vi "Toast With Multiple Actions.vi"(8 "error in":errorcluster) -> (0 "error out":errorcluster, 3 "Toast XML":string)   [LabVIEW 2026]
doc: "Distinguish clicks on the Accept button, Reject button and toast body. Inspect Activation.Arguments after each action. User Inputs is empty because the toast has no input field. Press Stop to close the example."
uses:
  ToastNotification/Activation.ctl
  ToastNotification/Argument.ctl
  PlugIns/UserEventActivationHandler/UserEventActivationHandler.lvclass
  PlugIns/UserEventActivationHandler/UserEventActivationHandler.lvclass/UserEventActivationHandler.ctl
  PlugIns/UserEventActivationHandler/Read Event Ref.vi
  ToastBuilder/ToastBuilder.lvclass
  ToastBuilder/Create ToastBuilder.vi
  ToastService/ToastService.lvclass
  ToastNotification/ToastNotification.lvlib
panel:
  out "error":errorcluster
  out "Activation":T1
  in  "stop":bool
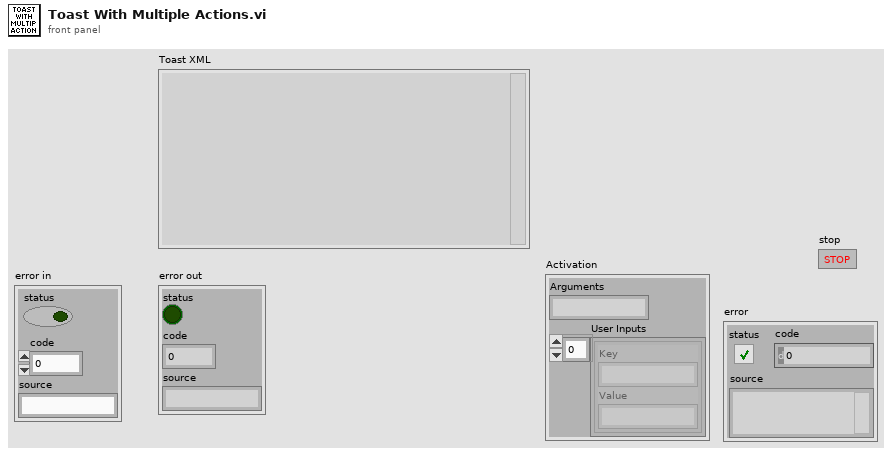
[diagram p1: front panel]
types:
  T1 = typedef "ToastNotification.lvlib/Activation.ctl" = cluster{"Arguments":string, "User Inputs":T2[]}
  T2 = typedef "ToastNotification.lvlib/Argument.ctl" = cluster{"Key":string, "Value":string}
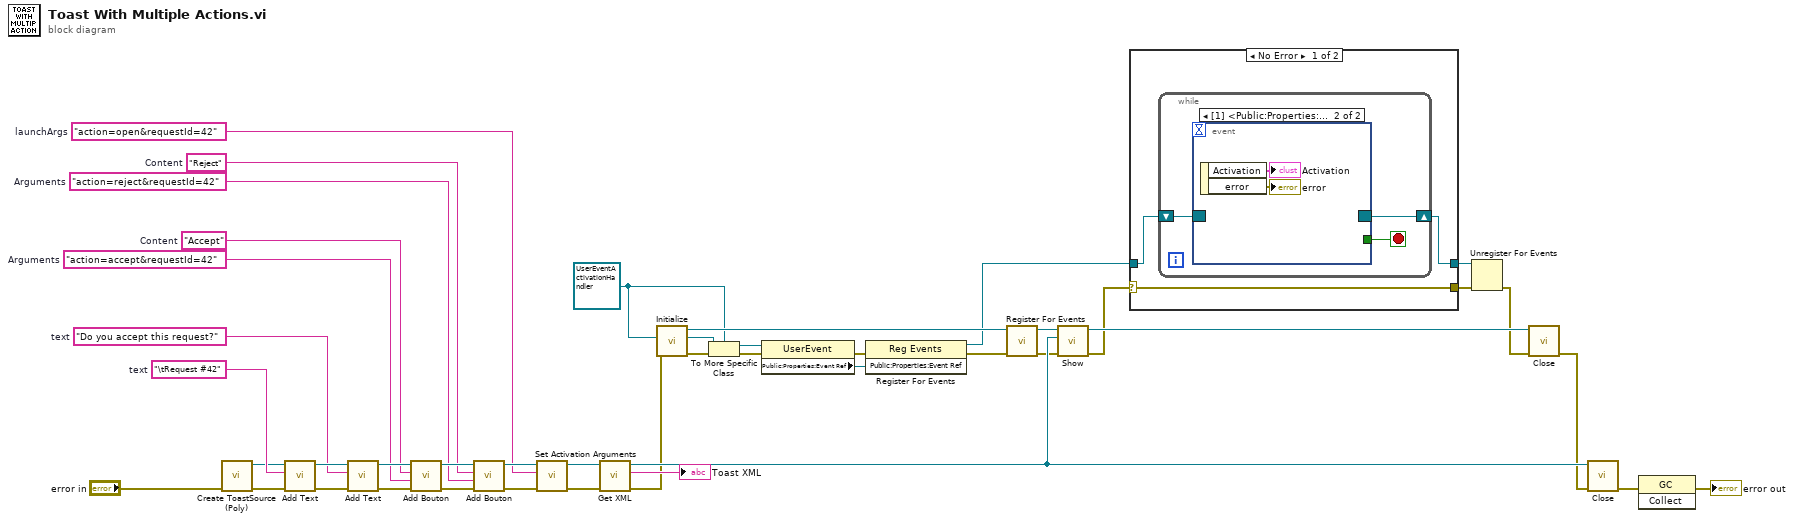
[diagram p0: block diagram]
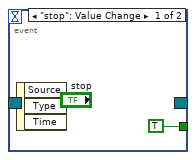
[diagram p2: hidden frame]
diagram:
  w1 = "action=open&requestId=42"  # launchArgs
  w10 = "action=reject&requestId=42"  # Arguments
  w9 = "Reject"  # Content
  w11 = "action=accept&requestId=42"  # Arguments
  w12 = "Accept"  # Content
  w13 = "Do you accept this request?"  # text
  w14 = "\tRequest #42"  # text
  w31 = refnum<class "UserEventActivationHandler.lvclass"> refnum
  n1 = call-poly "Create ToastSource (Poly).vi"("error in"="error in") -> ("error out"=w7:errorcluster, "ToastBuilder out"=w8:refnum<class "ToastBuilder.lvclass">)  [unwired: 9 in]
  n2 = call "Add Text.vi"("error in"=w7, "text"=w14, "ToastBuilder in"=w8) -> ("error out"=w19:errorcluster, "ToastBuilder out"=w20:refnum<class "ToastBuilder.lvclass">)  [unwired: 7 in]
  n3 = call "Add Text.vi"("error in"=w19, "text"=w13, "ToastBuilder in"=w20) -> ("error out"=w17:errorcluster, "ToastBuilder out"=w18:refnum<class "ToastBuilder.lvclass">)  [unwired: 7 in]
  n4 = call "Add Bouton.vi"("error in (no error)"=w17, "Arguments"=w11, "Content"=w12, "ToastBuilder in"=w18) -> ("error out"=w15:errorcluster, "ToastBuilder out"=w16:refnum<class "ToastBuilder.lvclass">)  [unwired: 6 in]
  n5 = call "Add Bouton.vi"("error in (no error)"=w15, "Arguments"=w10, "Content"=w9, "ToastBuilder in"=w16) -> ("error out"=w5:errorcluster, "ToastBuilder out"=w3:refnum<class "ToastBuilder.lvclass">)  [unwired: 6 in]
  n6 = call "Set Activation Arguments.vi"("error in (no error)"=w5, "launchArgs"=w1, "ToastBuilder in"=w3) -> ("error out"=w4:errorcluster, "ToastBuilder out"=w2:refnum<class "ToastBuilder.lvclass">)  [unwired: 7 in]
  n7 = call-dynamic "Get XML.vi"("error in"=w4, "ToastBuilder in"=w2) -> ("error out"=w40:errorcluster, "GetContent"=→"Toast XML":string, "ToastBuilder out"=w41:refnum<class "ToastBuilder.lvclass">)  [unwired: 7 in]
  n8 = call "Initialize.vi"("error in (no error)"=w40, "ActivationHandler in"=w31) -> ("error out"=w38:errorcluster, "ActivationHandler out"=w30:refnum<class "UserEventActivationHandler.lvclass">, "ToastService out"=w36:refnum<class "ToastService.lvclass">)  [unwired: 7 in]
  n9 = To More Specific Class(target class=w31, reference=w30, error in=w38) -> (specific class reference=w27:refnum<class "UserEventActivationHandler.lvclass">, error out=w29:errorcluster)
  n10 = property class="UserEvent"(reference=w27, error in=w29) -> (error out=w28:errorcluster, "Public:Properties:Event Ref"=w26:refnum<user-event>)  [unwired: 1 out]
  n11 = register-events(error in=w28, w26) -> (reference out=w25:refnum<event-registration>, error out=w23:errorcluster)  [unwired: 1 in]
  n12 = call "Register For Events.vi"("error in (no error)"=w23, "ToastService in"=w36) -> ("error out"=w37:errorcluster, "ToastService out"=w35:refnum<class "ToastService.lvclass">)  [unwired: 8 in]
  n13 = call "Show.vi"("error in (no error)"=w37, "ToastSource in"=w41, "ToastService in"=w35) -> ("error out"=w6:errorcluster, "ToastService out"=w34:refnum<class "ToastService.lvclass">)  [unwired: 7 in]
  n14 = case shown="No Error" w6 {
    selector: w6 -> [w44 w54]
    tunnel: w25 -> [w46 w53]
    tunnel: [w45 w53] -> w24
    tunnel: [w44 w54] -> w22
    frame No Error {
      n15 = while {
        shift-right: [w48] -> w45
        shift-left: w46 -> [w49]
        stop <- w47 stop-if-true
        n16 = event shown="[1] <Public:Properties:Event Ref>: User Event" {
          selector: w49 -> [_ _]
          dyn-events: [_ _] -> w48
          timeout: _ -> [_ _]
          tunnel: [TRUE _] -> w47
          event "stop": Value Change {
            n17 = event-data() -> ()  [unwired: 1 in, 3 out]
          }
          event User Event {
            n18 = event-data() -> ("Activation"=→"Activation":T1, "error"=→"error":errorcluster)  [unwired: 1 in]
          }
        }
      }
    }
    frame Error {
    }
  }
  n19 = Unregister For Events(event registration refnum=w24, error in=w22) -> (error out=w21:errorcluster)
  n20 = call "Close.vi"("error in (no error)"=w21, "ToastService in"=w34) -> ("error out"=w39:errorcluster)  [unwired: 9 in]
  n21 = call-dynamic "Close.vi"("error in"=w39, "ToastBuilder in"=w41) -> ("error out"=w33:errorcluster)  [unwired: 9 in]
  n22 = invoke class="GC" method="Collect"(error in=w33) -> (error out=→"error out":errorcluster)  [unwired: 2 in, 2 out]
